vi "Untitled 1.vi"   [LabVIEW 2025]
uses:
  <vilib>/MakerHub/Leap/LMH-Leap.lvlib
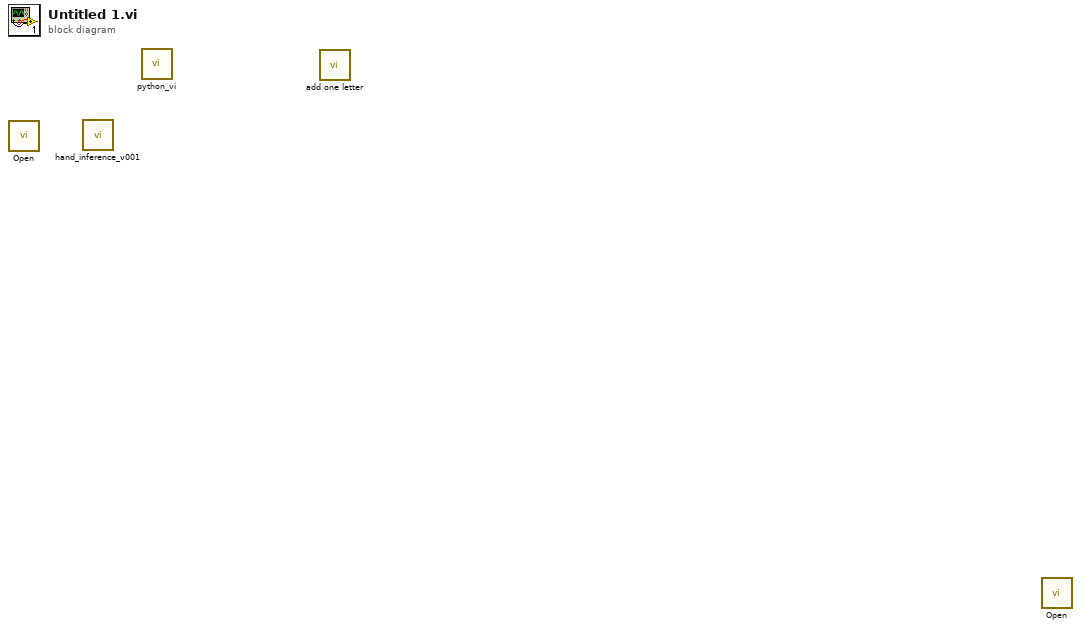
[diagram p0: block diagram]
diagram:
  n1 = call <vilib>:"Open.vi"() -> ()  [unwired: 10 in, 2 out]
  n2 = call "hand_inference_v001.vi"() -> ()  [unwired: 12 in]
  n3 = call "python_vi.vi"() -> ()  [unwired: 12 in]
  n4 = call "add one letter.vi"() -> ()  [unwired: 12 in]
  n5 = call <vilib>:"Open.vi"() -> ()  [unwired: 10 in, 2 out]
